vi "ReadDIOData.vi"(8 "error in (no error)":errorcluster, 11 "object in":refnum<class "DIO-Configuration.lvclass">) -> (0 "error out":errorcluster, 2 "Data":T1, 3 "object out":refnum<class "DIO-Configuration.lvclass">)   [LabVIEW 2021, in "DIO-Configuration.lvclass"]
uses:
  DIO-Configuration.lvclass
  tdef/Data.ctl
  Device Channels/DAQmx/DIO-Configuration_class/tdef/Direction.ctl
  DIO-Configuration.lvclass/DIO-Configuration.ctl
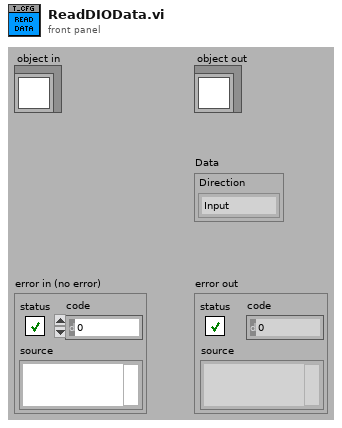
[diagram p1: front panel]
types:
  T1 = typedef "DIO-Configuration.lvclass/Data.ctl" = cluster{"Direction":T2}
  T2 = typedef "DIO-Configuration.lvclass/Direction.ctl" = enum16{"Input", "Output"}
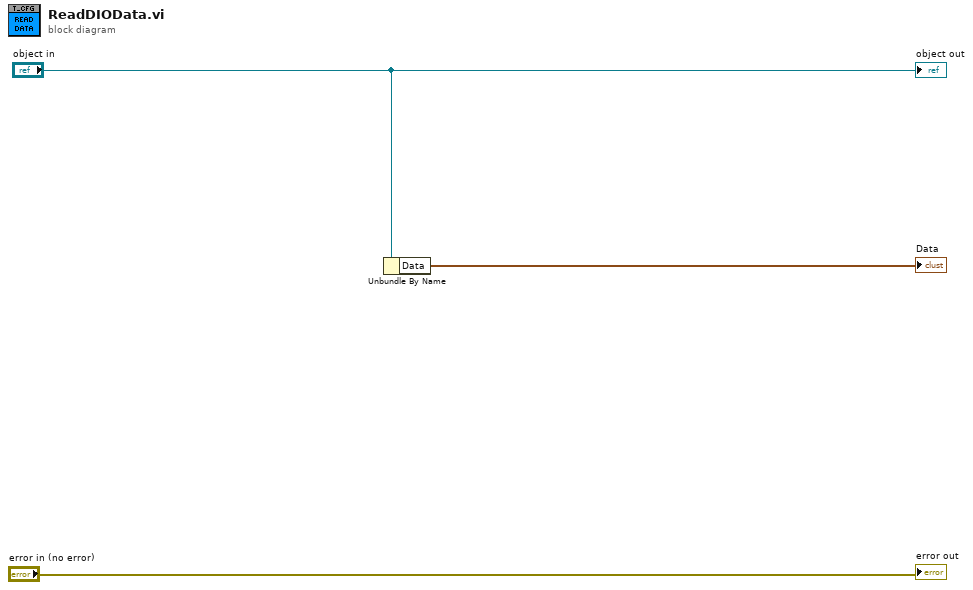
[diagram p0: block diagram]
diagram:
  n1 = Unbundle By Name("object in") -> ("Data"=→"Data":T1)
  "error out" <- "error in (no error)"
  "object out" <- "object in"
